vi "[ex ce] Tank Simulator.vi"() -> ()   [LabVIEW 2021]
doc: "<B>Varible Manager example</B>\n\nThis example demonstrates a use of variable histories and aliases. It consists of two top-level VIs (when you run this VI, both the VIs will be launched):\n\n1) <B>[ex ce] Tank Simulator.vi</B> simulates a tank with inlet and outlet pipes. It creates a variable context with some variables to store parameters of work. Every variable gets a history attached and an alias. When the VI writes a variable value, the variable history is automatically updated.\n\n2) <B>[ex ce] Tank Parameters History.vi</B> reads history of the variables written by the previous VI and displays it on graphs. To access the variables, this VI uses their known aliases. This method makes it possible to access variables without a need to know a variable context where the variables reside.\n\n::: CalcExpress Toolkit :::\nCopyright (c) 2000-2026 Konstantin Shifershteyn. All rights reserved."
panel:
  in  "local stop":bool
  in  "History length":i32=1000 min=100 max=1000
  out "Volume":dbl(slide) min=0.0 scale=0.0..1000.0 scale format="%.1f"
  in  "Pipe capacity":dbl=25.0 format="%.2f"
  in  "Pump capacity":dbl=50.0 format="%.2f"
  in  "stop":bool
  out "Pump":u16(ring)
  out "Outflow Rate":dbl format="%.2f"
  # "This example consists of two top-level VIs:\n  [ex ce] Tank Simulator.vi  and\n  [ex ce] Tank Parameters History.vi\nWhen you start this VI, both the VIs are launched."
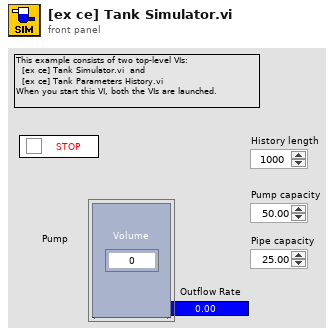
[diagram p1: front panel]
types:
  T1 = enum32{"nothing", "reset", "assign name", "get name", "get handle"}
  T2 = typedef "VarMan Variable Context Handle.ctl" = i32
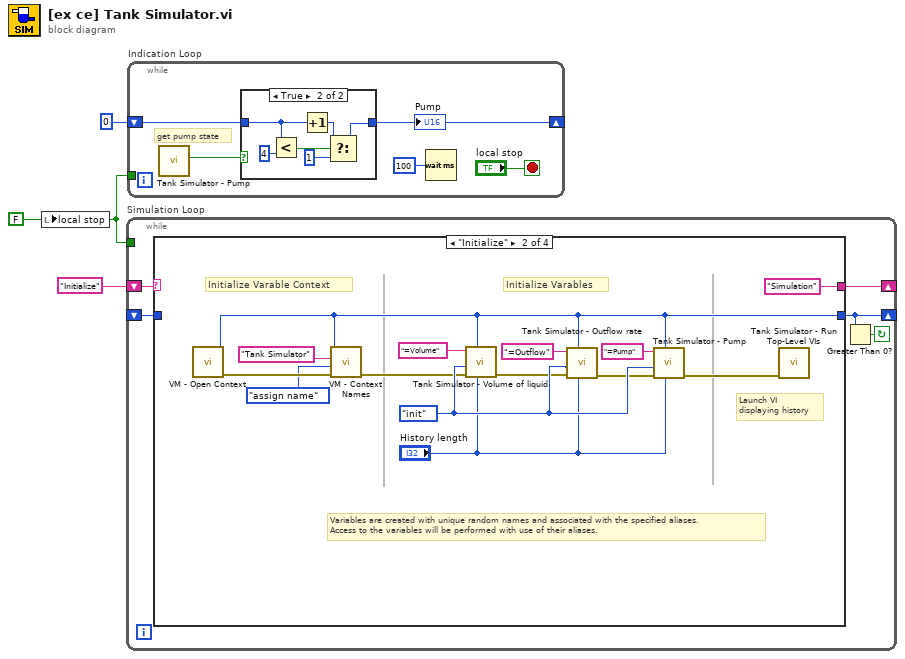
[diagram p0: block diagram]
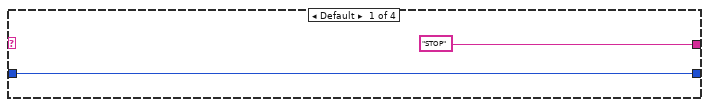
[diagram p2: hidden frame]
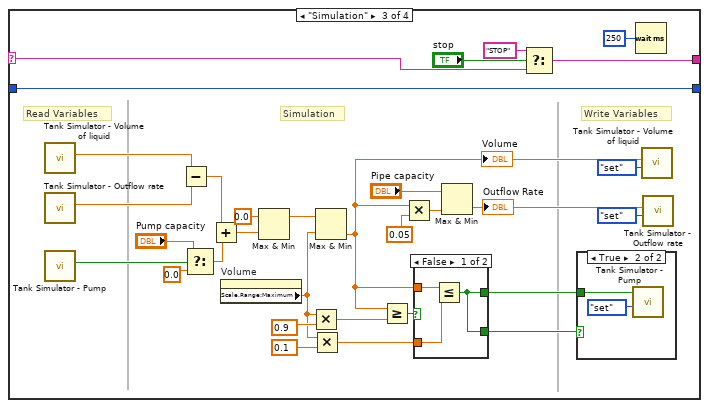
[diagram p3: hidden frame]
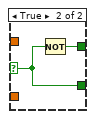
[diagram p5: hidden frame]
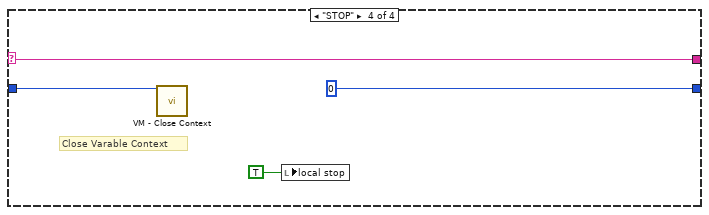
[diagram p6: hidden frame]
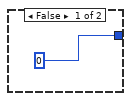
[diagram p7: hidden frame]
diagram:
  w2 = FALSE ("local stop")
  n1 = local write "local stop"(w2) -> ()
  n2 = while "Simulation Loop" {
    tunnel: w2 -> [_]
    shift-left: _ -> [w6]
    shift-right: [w4] -> _
    shift-left: "Initialize" -> [w8]
    shift-right: [w7] -> _
    stop <- w5 continue-if-true
    n3 = case shown="\"Initialize\"" w8 {
      selector: w8 -> [_ _ w27 w65]
      tunnel: ["STOP" ("t") "Simulation" w32 w65] -> w7
      tunnel: [w10 w12 w30 0 ("VC Handle out")] -> w4
      tunnel: w6 -> [w10 _ w30 w66]
      frame Default {
      }
      frame "Initialize" {
        w23 = enum16{"init", "get", "set"}."init" ("cmd")
        # "Variables are created with unique random names and associated with the specified aliases.\nAccess to the variables will be performed with use of their aliases."
        # "Launch VI\ndisplaying history"
        # "Initialize Varables"
        # "Initialize Varable Context"
        n4 = call "VM - Open Context.vi"() -> ("error out"=w17:errorcluster, "VC Handle out"=w12:T2)  [unwired: 9 in, 1 out]
        n5 = call "VM - Context Names.vi"("error in"=w17, "action"=T1."assign name", "VC Name"="Tank Simulator", "VC Handle"=w12) -> ("error out"=w18:errorcluster)  [unwired: 2 in, 3 out]
        n6 = call "Tank Simulator - Volume of liquid.vi"("history length"="History length", "VC Handle"=w12, "error in"=w18, "cmd"=w23, "var name"="=Volume") -> ("error out"=w19:errorcluster)  [unwired: 3 in, 3 out]
        n7 = call "Tank Simulator - Outflow rate.vi"("history length"="History length", "VC Handle"=w12, "error in"=w19, "cmd"=w23, "var name"="=Outflow") -> ("error out"=w22:errorcluster)  [unwired: 3 in, 3 out]
        n8 = call "Tank Simulator - Pump.vi"("history length"="History length", "VC Handle"=w12, "error in"=w22, "cmd"=w23, "var name"="=Pump") -> ("error out"=w11:errorcluster)  [unwired: 3 in, 3 out]
        n9 = call "Tank Simulator - Run Top-Level VIs.vi"("error in (no error)"=w11) -> ()  [unwired: 8 in, 1 out]
      }
      frame "Simulation" {
        # "Write Variables"
        # "Simulation"
        # "Read Variables"
        n10 = call "Tank Simulator - Volume of liquid.vi"() -> ("value out"=w54:dbl)  [unwired: 8 in, 3 out]
        n11 = call "Tank Simulator - Outflow rate.vi"() -> ("value out"=w41:dbl)  [unwired: 8 in, 3 out]
        n12 = call "Tank Simulator - Pump.vi"() -> ("state out"=w39:bool)  [unwired: 8 in, 3 out]
        n13 = Subtract(x=w54, y=w41) -> (x-y=w55:dbl)
        n14 = Select(t="Pump capacity", s=w39, f=0.0) -> (s? t:f=w36:dbl)
        n15 = Add(x=w55, y=w36) -> (x+y=w53:dbl)
        n16 = property on="Volume" class="Slide (strict)"() -> ("Scale.Range:Maximum"=w28:dbl)  [unwired: 2 in, 2 out]
        n17 = Max & Min(x=0.0 ("t"), y=w53) -> (max(x,y)=w29:dbl)  [unwired: 1 out]
        n18 = Multiply(x=w28, y=0.9) -> (x*y=w48:dbl)
        n19 = Multiply(x=w28, y=0.1) -> (x*y=w44:dbl)
        n20 = Max & Min(x=w29, y=w28) -> (min(x,y)=w25:dbl)  [unwired: 1 out]
        "Volume" <- w25
        n21 = Greater Or Equal?(x=w25, y=w48) -> (x >= y?=w51:bool)
        n22 = Multiply(x=w25, y=0.05) -> (x*y=w35:dbl)
        n23 = case shown="False" w51 {
          selector: w51 -> [_ w62]
          tunnel: w25 -> [w60 _]
          tunnel: [w59 w61] -> w49
          tunnel: [w59 w62] -> w50
          tunnel: w44 -> [w58 _]
          frame False {
            n24 = Less Or Equal?(x=w60, y=w58) -> (x <= y?=w59:bool)
          }
          frame True {
            n25 = Not(x=w62) -> (.not. x?=w61:bool)
          }
        }
        n26 = Max & Min(x="Pipe capacity", y=w35) -> (min(x,y)=w26:dbl)  [unwired: 1 out]
        "Outflow Rate" <- w26
        n27 = Select(t="STOP", s="stop", f=w27) -> (s? t:f=w32:string)
        n28 = case shown="True" w50 {
          tunnel: w49 -> [_ w57]
          frame False {
          }
          frame True {
            n29 = call "Tank Simulator - Pump.vi"("cmd"=enum16{"init", "get", "set"}."set", "state in"=w57) -> ()  [unwired: 6 in, 4 out]
          }
        }
        n30 = Wait (ms)(milliseconds to wait=u32 250) -> ()  [unwired: 1 out]
        n31 = call "Tank Simulator - Volume of liquid.vi"("cmd"=enum16{"init", "get", "set"}."set", "value in"=w25) -> ()  [unwired: 6 in, 4 out]
        n32 = call "Tank Simulator - Outflow rate.vi"("cmd"=enum16{"init", "get", "set"}."set", "value in"=w26) -> ()  [unwired: 6 in, 4 out]
      }
      frame "STOP" {
        # "Close Varable Context"
        n33 = call "VM - Close Context.vi"("VC Handle"=w66) -> ()  [unwired: 9 in, 2 out]
        n34 = local write "local stop"(TRUE ("local stop")) -> ()
      }
    }
    n35 = Greater Than 0?(x=w4) -> (x > 0?=w5:bool)
  }
  n36 = while "Indication Loop" {
    tunnel: w2 -> [_]
    shift-right: [w67] -> _
    shift-left: u16 0 ("Pump") -> [w68]
    stop <- "local stop" stop-if-true
    # "get pump state"
    n37 = call "Tank Simulator - Pump.vi"() -> ("state out"=w71:bool)  [unwired: 8 in, 3 out]
    n38 = case shown="True" w71 {
      tunnel: [u16 0 w77] -> w67
      tunnel: w68 -> [_ w73]
      frame False {
      }
      frame True {
        n39 = Less?(x=w73, y=u16 4) -> (x < y?=w78:bool)
        n40 = Increment(x=w73) -> (x+1=w76:u16)
        n41 = Select(t=w76, s=w78, f=u16 1) -> (s? t:f=w77:u16)
      }
    }
    "Pump" <- w67
    n42 = Wait (ms)(milliseconds to wait=u32 100) -> ()  [unwired: 1 out]
  }
